vi "get TurnTable Parameter.vi"(8 "error in (no error)":errorcluster caption="에러 입력(에러 없음)", 11 "Interface - Turn Table 입력":refnum<class "Interface - Turn Table.lvclass">) -> (0 "error out":errorcluster caption="에러 출력", 2 "Turn Table Info":T1 {"Target Angle" min=0.0 max=360.0}, 3 "Interface - Turn Table 출력":refnum<class "Interface - Turn Table.lvclass">)   [LabVIEW 2023, in "Turn Table and Mast.lvlib" / "Interface - Turn Table.lvclass"]
uses:
  Interface - Turn Table.lvclass
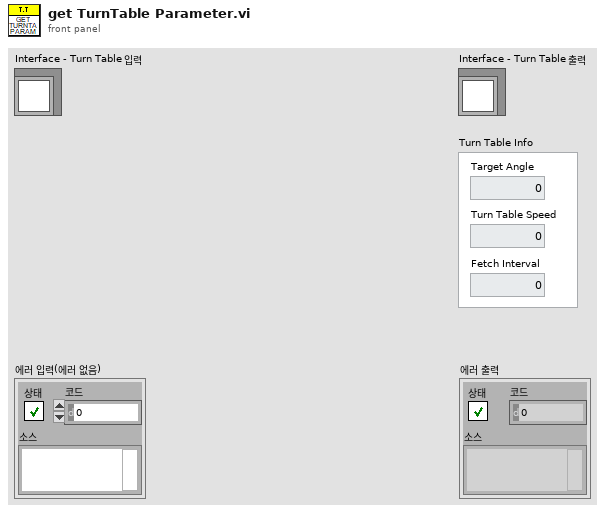
[diagram p1: front panel]
types:
  T1 = cluster{"Target Angle":dbl, "Turn Table Speed":i32, "Fetch Interval":i32}
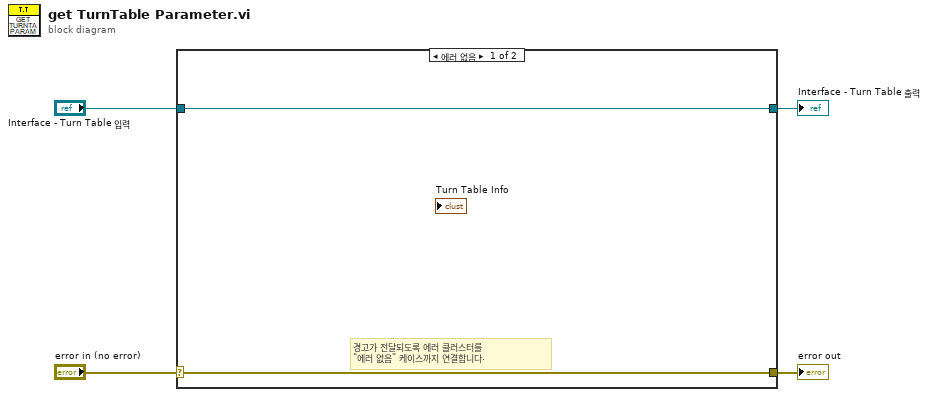
[diagram p0: block diagram]
diagram:
  n1 = case shown="에러 없음" "error in (no error)" {
    selector: "error in (no error)" -> [w5 w8]
    tunnel: [w5 w8] -> w3
    tunnel: [w6 w7] -> w1
    tunnel: "Interface - Turn Table 입력" -> [w6 w7]
    frame No Error {
      # "경고가 전달되도록 에러 클러스터를\n\"에러 없음\" 케이스까지 연결합니다."
    }
    frame Error {
    }
  }
  "error out" <- w3
  "Interface - Turn Table 출력" <- w1
